vi "Arret acquisitions.vi"() -> ()   [LabVIEW 2022 SP3]
panel:
  in  "Bouton Annuler":bool
  out "attente depuis (s)":i64
  # "Arrêt des acquisitions\nen cours\nVeuillez patienter"
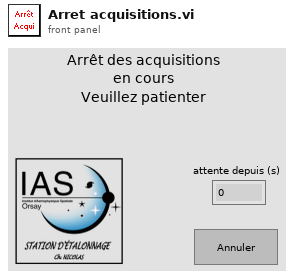
[diagram p1: front panel]
types:
  T1 = enum32{"Bad", "Idle", "Run top level", "Running"}
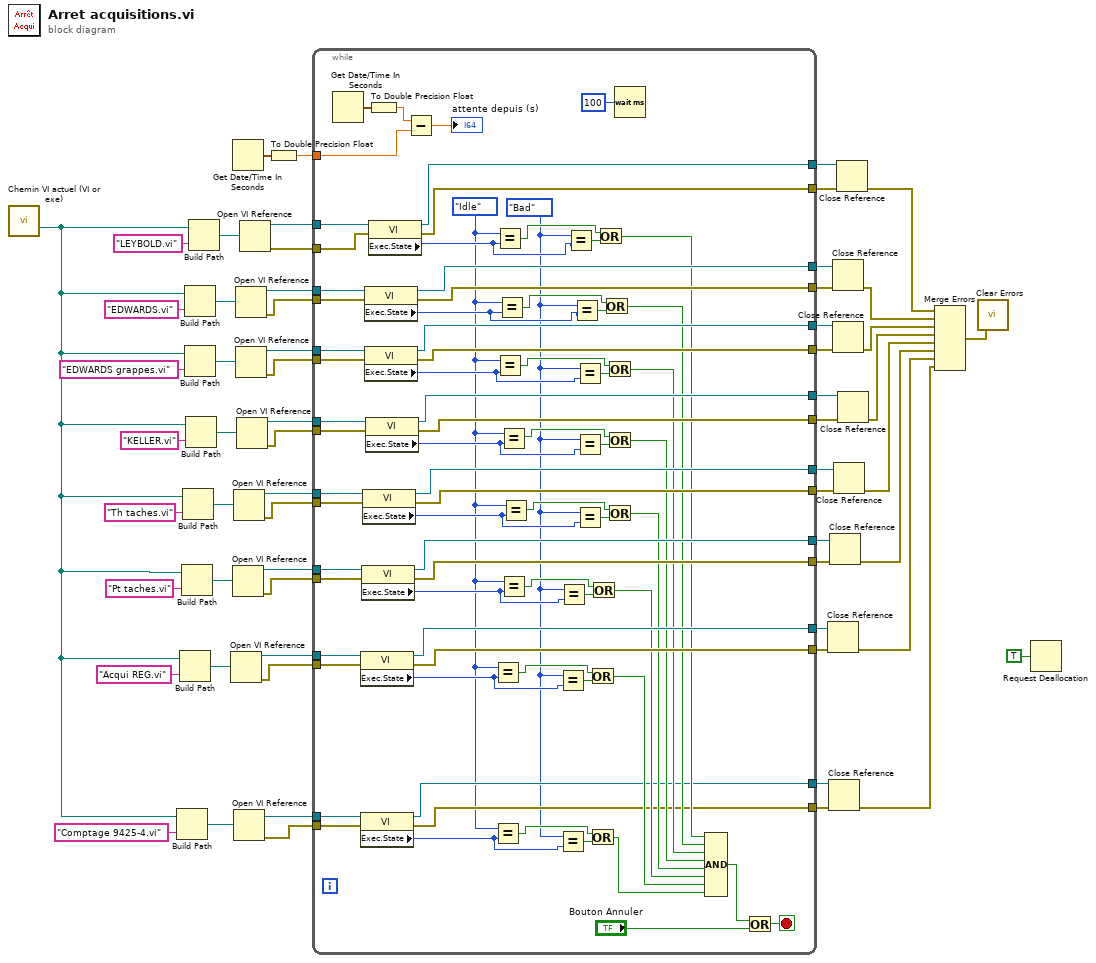
[diagram p0: block diagram]
diagram:
  n1 = call "Chemin VI actuel (VI or exe).vi"() -> ("VI or executable installation directory"=w1:path)  [unwired: 14 in, 1 out]
  n2 = Build Path(base path=w1, name or relative path="Comptage 9425-4.vi" ("nom ou chemin relatif")) -> (appended path=w8:path)
  n3 = Build Path(base path=w1, name or relative path="Acqui REG.vi" ("nom ou chemin relatif")) -> (appended path=w20:path)
  n4 = Build Path(base path=w1, name or relative path="Pt taches.vi" ("nom ou chemin relatif")) -> (appended path=w55:path)
  n5 = Build Path(base path=w1, name or relative path="Th taches.vi" ("nom ou chemin relatif")) -> (appended path=w52:path)
  n6 = Build Path(base path=w1, name or relative path="EDWARDS.vi" ("nom ou chemin relatif")) -> (appended path=w46:path)
  n7 = Build Path(base path=w1, name or relative path="EDWARDS grappes.vi" ("nom ou chemin relatif")) -> (appended path=w14:path)
  n8 = Build Path(base path=w1, name or relative path="KELLER.vi" ("nom ou chemin relatif")) -> (appended path=w49:path)
  n9 = Build Path(base path=w1, name or relative path="LEYBOLD.vi" ("nom ou chemin relatif")) -> (appended path=w43:path)
  n10 = Open VI Reference(vi path=w20) -> (vi reference=w18:refnum<vi>, error out=w19:errorcluster)  [unwired: 5 in]
  n11 = Get Date/Time In Seconds() -> (seconds since 1Jan1904=w41:timestamp)
  n12 = Open VI Reference(vi path=w55) -> (vi reference=w61:refnum<vi>, error out=w56:errorcluster)  [unwired: 5 in]
  n13 = Open VI Reference(vi path=w52) -> (vi reference=w51:refnum<vi>, error out=w57:errorcluster)  [unwired: 5 in]
  n14 = Open VI Reference(vi path=w8) -> (vi reference=w6:refnum<vi>, error out=w5:errorcluster)  [unwired: 5 in]
  n15 = Open VI Reference(vi path=w46) -> (vi reference=w45:refnum<vi>, error out=w59:errorcluster)  [unwired: 5 in]
  n16 = Open VI Reference(vi path=w14) -> (vi reference=w15:refnum<vi>, error out=w12:errorcluster)  [unwired: 5 in]
  n17 = Open VI Reference(vi path=w49) -> (vi reference=w50:refnum<vi>, error out=w58:errorcluster)  [unwired: 5 in]
  n18 = Open VI Reference(vi path=w43) -> (vi reference=w44:refnum<vi>, error out=w60:errorcluster)  [unwired: 5 in]
  n19 = To Double Precision Float(number=w41) -> (double precision float=w40:dbl)
  n20 = while {
    tunnel: w61 -> [w135]
    tunnel: w60 -> [w134]
    tunnel: w59 -> [w133]
    tunnel: w58 -> [w132]
    tunnel: w57 -> [w131]
    tunnel: w56 -> [w130]
    tunnel: w51 -> [w129]
    tunnel: w50 -> [w128]
    tunnel: w45 -> [w127]
    tunnel: w44 -> [w119]
    tunnel: w40 -> [w124]
    tunnel: [w118] -> w39
    tunnel: [w117] -> w38
    tunnel: [w116] -> w37
    tunnel: [w115] -> w36
    tunnel: [w114] -> w34
    tunnel: [w113] -> w35
    tunnel: [w112] -> w33
    tunnel: [w111] -> w32
    tunnel: [w110] -> w30
    tunnel: [w109] -> w31
    tunnel: w18 -> [w105]
    tunnel: w19 -> [w106]
    tunnel: [w107] -> w23
    tunnel: [w108] -> w22
    tunnel: w12 -> [w102]
    tunnel: w15 -> [w103]
    tunnel: [w101] -> w11
    tunnel: [w100] -> w10
    tunnel: w6 -> [w68]
    tunnel: w5 -> [w67]
    tunnel: [w65] -> w4
    tunnel: [w64] -> w3
    stop <- w120 stop-if-true
    w62 = T1."Bad" ("Exécution : état")
    w63 = T1."Idle" ("Exécution : état")
    n21 = Get Date/Time In Seconds() -> (seconds since 1Jan1904=w126:timestamp)
    n22 = property class="VI"(reference=w105, error in=w106) -> (reference out=w107:refnum<vi>, error out=w108:errorcluster, "Exec.State"=w73:T1)
    n23 = property class="VI"(reference=w68, error in=w67) -> (reference out=w65:refnum<vi>, error out=w64:errorcluster, "Exec.State"=w70:T1)
    n24 = property class="VI"(reference=w135, error in=w130) -> (reference out=w110:refnum<vi>, error out=w109:errorcluster, "Exec.State"=w77:T1)
    n25 = property class="VI"(reference=w129, error in=w131) -> (reference out=w112:refnum<vi>, error out=w111:errorcluster, "Exec.State"=w81:T1)
    n26 = property class="VI"(reference=w127, error in=w133) -> (reference out=w116:refnum<vi>, error out=w115:errorcluster, "Exec.State"=w93:T1)
    n27 = property class="VI"(reference=w103, error in=w102) -> (reference out=w101:refnum<vi>, error out=w100:errorcluster, "Exec.State"=w89:T1)
    n28 = property class="VI"(reference=w128, error in=w132) -> (reference out=w114:refnum<vi>, error out=w113:errorcluster, "Exec.State"=w85:T1)
    n29 = To Double Precision Float(number=w126) -> (double precision float=w125:dbl)
    n30 = property class="VI"(reference=w119, error in=w134) -> (reference out=w118:refnum<vi>, error out=w117:errorcluster, "Exec.State"=w97:T1)
    n31 = Subtract(x=w125, y=w124) -> (x-y=→"attente depuis (s)":dbl)
    n32 = Equal?(x=w63, y=w73) -> (x = y?=w72:bool)
    n33 = Equal?(x=w63, y=w70) -> (x = y?=w71:bool)
    n34 = Equal?(x=w63, y=w97) -> (x = y?=w96:bool)
    n35 = Equal?(x=w63, y=w89) -> (x = y?=w88:bool)
    n36 = Equal?(x=w63, y=w93) -> (x = y?=w94:bool)
    n37 = Equal?(x=w63, y=w85) -> (x = y?=w84:bool)
    n38 = Equal?(x=w63, y=w77) -> (x = y?=w76:bool)
    n39 = Equal?(x=w63, y=w81) -> (x = y?=w80:bool)
    n40 = Equal?(x=w62, y=w73) -> (x = y?=w75:bool)
    n41 = Equal?(x=w62, y=w70) -> (x = y?=w69:bool)
    n42 = Equal?(x=w62, y=w77) -> (x = y?=w79:bool)
    n43 = Equal?(x=w62, y=w97) -> (x = y?=w99:bool)
    n44 = Equal?(x=w62, y=w93) -> (x = y?=w95:bool)
    n45 = Equal?(x=w62, y=w89) -> (x = y?=w91:bool)
    n46 = Equal?(x=w62, y=w85) -> (x = y?=w87:bool)
    n47 = Equal?(x=w62, y=w81) -> (x = y?=w83:bool)
    n48 = Or(x=w72, y=w75) -> (x .or. y?=w74:bool)
    n49 = Or(x=w71, y=w69) -> (x .or. y?=w66:bool)
    n50 = Or(x=w76, y=w79) -> (x .or. y?=w78:bool)
    n51 = Or(x=w96, y=w99) -> (x .or. y?=w98:bool)
    n52 = Or(x=w94, y=w95) -> (x .or. y?=w92:bool)
    n53 = Or(x=w88, y=w91) -> (x .or. y?=w90:bool)
    n54 = Or(x=w84, y=w87) -> (x .or. y?=w86:bool)
    n55 = Or(x=w80, y=w83) -> (x .or. y?=w82:bool)
    n56 = Wait (ms)(milliseconds to wait=u32 100 ("attente (ms)")) -> ()  [unwired: 1 out]
    n57 = Compound Arithmetic op=AND(w98, w92, w90, w86, w82, w78, w74, w66) -> (w122:bool)
    n58 = Or(x=w122, y="Bouton Annuler") -> (x .or. y?=w120:bool)
  }
  n59 = Close Reference(reference=w23, error in (no error)=w22) -> (error out=w17:errorcluster)
  n60 = Close Reference(reference=w4, error in (no error)=w3) -> (error out=w2:errorcluster)
  n61 = Close Reference(reference=w30, error in (no error)=w31) -> (error out=w25:errorcluster)
  n62 = Close Reference(reference=w37, error in (no error)=w36) -> (error out=w28:errorcluster)
  n63 = Close Reference(reference=w11, error in (no error)=w10) -> (error out=w9:errorcluster)
  n64 = Close Reference(reference=w33, error in (no error)=w32) -> (error out=w26:errorcluster)
  n65 = Close Reference(reference=w39, error in (no error)=w38) -> (error out=w29:errorcluster)
  n66 = Close Reference(reference=w34, error in (no error)=w35) -> (error out=w27:errorcluster)
  n67 = Merge Errors(w29, w28, w9, w27, w26, w25, w17, w2) -> (w24:errorcluster)
  n68 = call <vilib>:"Clear Errors.vi"("error in (no error)"=w24) -> ()  [unwired: 5 in, 2 out]
  n69 = Request Deallocation(TRUE ("flag")) -> ()
